vi "Host Image Acquisition Module.vi"(8 "error in":errorcluster, 11 "Operation":T3) -> (0 "error out":errorcluster, 1 "Image Acquired":bool, 2 "Acq In Progress":bool, 3 "Image":T2(plugin-control))   [LabVIEW 2013]
uses:
  Host Image Acquisition Module Enum.ctl
  Acquisition Settings Cluster.ctl
  <vilib>/vision/Image Controls.llb/IMAQ Image.ctl
  Common/CL Configuration.ctl
  Common/CL Signal Mapping.ctl
  Image Acquisition Settings FG Enum.ctl
  System Status/Status FG Enum.ctl
  Image Processing/Mask ROI FG Enum.ctl
  <vilib>/rvi/interface/common/niFpgaWaitOnOcc.vi
  <vilib>/FPGAPlugInAG/PCIe-1473R/niLvFpga_Reset_PCIe-1473R.vi
  <vilib>/Utility/error.llb/Error Cluster From Error Code.vi
  <vilib>/rvi/errors/niLvFpgaAdjustHostInterfaceError.vi
  <vilib>/FPGAPlugInAG/PCIe-1473R/niLvFpga_Run_PCIe-1473R.vi
  <vilib>/FPGAPlugInAG/PCIe-1473R/niLvFpga_Close_PCIe-1473R.vi
  <vilib>/rvi/interface/nirviMethod/nirviMethod.xnode
  FGs/FPGA_Reference.ctl
  8-Tap 8-bit Camera with DRAM Example/FPGA Bitfiles/8-Tap8-bitCamera_FPGATarget_8-Tap8-bit.lvbitx
  <vilib>/rvi/interface/nirviReadWriteControl/nirviReadWriteControl.xnode
  <vilib>/rvi/interface/nirviCloseFPGA/nirviCloseFPGA.xnode
  Common/Timing/Timing Lib.lvlib
  Globals/Average Sector Data.vi
  <vilib>/rvi/errors/niLvFpgaMergeErrorWithErrorCode.vi
  NiFpgaLv.dll
  <vilib>/FPGAPlugInAG/PCIe-1473R/niLvFpga_ReadFifo_PCIe-1473R.vi
  <vilib>/FPGAPlugInAG/PCIe-1473R/niLvFpga_ConfigureFifo_PCIe-1473R.vi
  <vilib>/FPGAPlugInAG/PCIe-1473R/niLvFpga_StartFifo_PCIe-1473R.vi
panel:
  out "Frames To Acquire":u32
  out "Image Height":u32
  out "Actual Depth":u32
  out "Target Sim TO":bool
  out "Cam Data Timeout":bool
  out "Sector FIFO Timeout":bool
  out "Host DMA Timeout":bool
  out "Number of Elements to Write Host DMA":u32
  out "Number of Elements to Read Cam Data":u32
  out "Image Data":u64[](array[numeric])
  out "Elements Remaining":u32
  out "Words per image":u32
  out "Num Frames read":u32
  out "DMA Words per Image":u32
  out "Acquire":bool
  in  "Acquisition Settings Cluster":T1={"Image Width"=1200, "Image Height"=788, "Frames To Acquire"=0, "Signal Mapping"=enum."Standard", "DMA Buffer Size\n(In Images)"=64} {"Image Height" max=65535; "Image Width" max=65535 step=40}
  out "Buffer Size":u32
  out "Acq'd Frame Width":u32=2040
  out "DMA Write Timeout":bool
  in  "Start Serial Server":bool
  out "Frames Acq'd":u32=1
  out "Acq'd Frame Height":u32=1088
  out "Initialized":bool
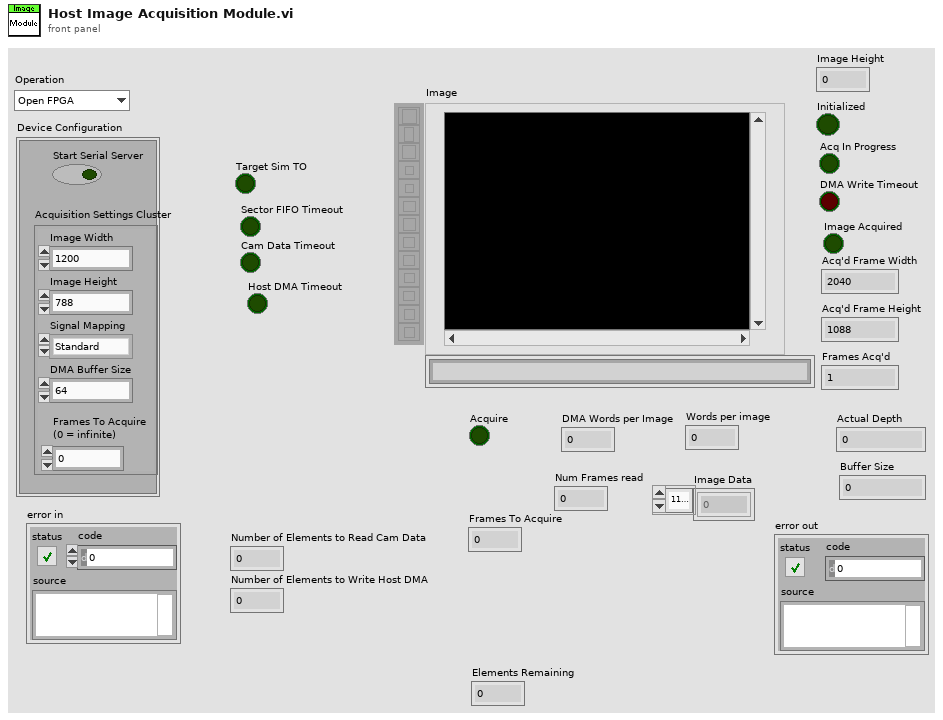
[diagram p1: front panel]
types:
  T1 = typedef "Acquisition Settings Cluster.ctl" = cluster{"Image Width":u32, "Image Height":u32, "Frames To Acquire":u32, "Signal Mapping":enum8{"Standard", "Basler 10-tap", "Vosskühler 10-tap"}, "DMA Buffer Size\n(In Images)":u32}
  T2 = typedef "IMAQ Image.ctl" = refnum<image>
  T3 = typedef "Host Image Acquisition Module Enum.ctl" = enum16{"Open FPGA", "Initialize DMA FIFO", "Load Sim Images", "Initialize Acquisition", "Update Sector Parameters", "Start Acquisition", "Aquire Image", "Read Averages", "Cancel Acquisition", "Close FPGA"}
  T4 = typedef "Image Acquisition Settings FG Enum.ctl" = enum16{"Read", "Write"}
  T5 = typedef "CL Signal Mapping.ctl" = enum8{"Standard", "Basler 10-tap", "Vosskühler 10-tap"}
  T6 = typedef "CL Configuration.ctl" = enum8{"Base", "Medium", "Full"}
  T7 = typedef "Status FG Enum.ctl" = enum16{"Reset", "Read", "Write"}
  T8 = typedef "Mask ROI FG Enum.ctl" = enum16{"Read", "Write"}
  T9 = enum16{"big-endian, network order", "native, host order", "little-endian"}
  T10 = typedef "FPGA_Reference.ctl" = refnum<k20>
  T11 = typedef "Image Type" = u32
  T12 = typedef "Mask ROI Cluster.ctl" = cluster{"left annulus":T13, "right annulus":T13, "Threshold Range":cluster{"Lower value":dbl, "Upper value":dbl}, "[Avg BG]":u8[], "Number of Sectors":u8, "Left ROI":T14, "Right ROI":T14, "Left Start Angle Duty Cycle":fxp<+,8,0>, "Left End Angle Duty Cycle":fxp<+,8,0>, "Right End Angle Duty Cycle":fxp<+,8,0>, "Right Start Angle Duty Cycle":fxp<+,8,0>, "[Sector ROIs]":T14[]}
  T13 = typedef "IMAQ Circle" = cluster{"Center X":i32, "Center Y":i32, "Inner Radius":i32, "Outer Radius":i32, "Start Angle":dbl, "End Angle":dbl}
  T14 = typedef "ROI Descriptor" = cluster{"Global Rectangle":i32[], "Contours":cluster{"ID":enum32{"External", "Internal"}, "Type":u32, "Coordinates":i32[]}[]}
  T15 = typedef "Sector Parameter Cluster.ctl" = cluster{"Start Angle":fxp<+/-,17,2>, "End Angle":fxp<+,17,3>, "Inner Radius":u16, "Outter Radius":u16, "Hinge X":u16, "Hinge Y":u16, "NumWingSectors":u8}
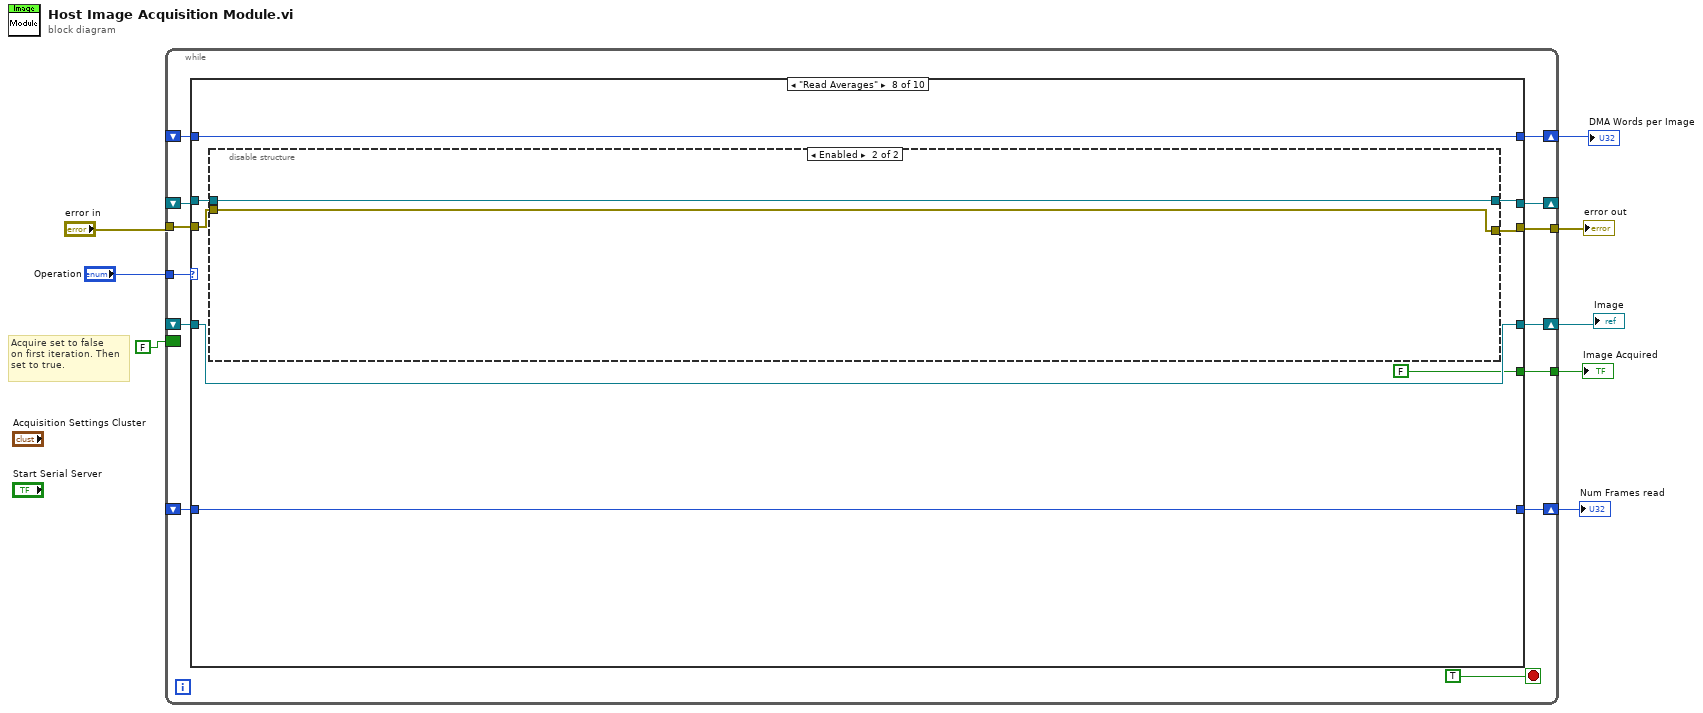
[diagram p0: block diagram]
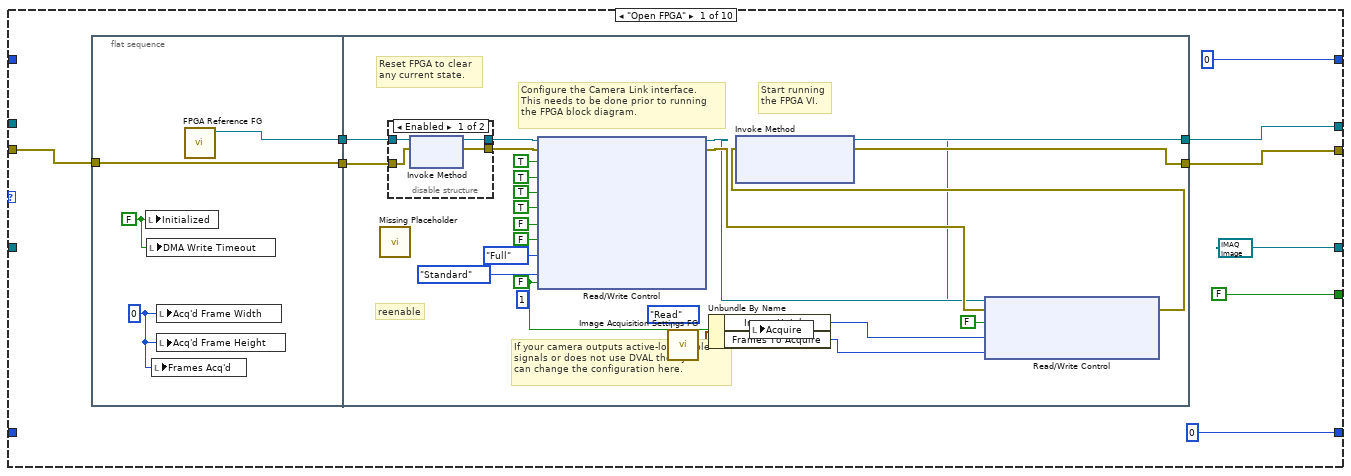
[diagram p2: hidden frame]
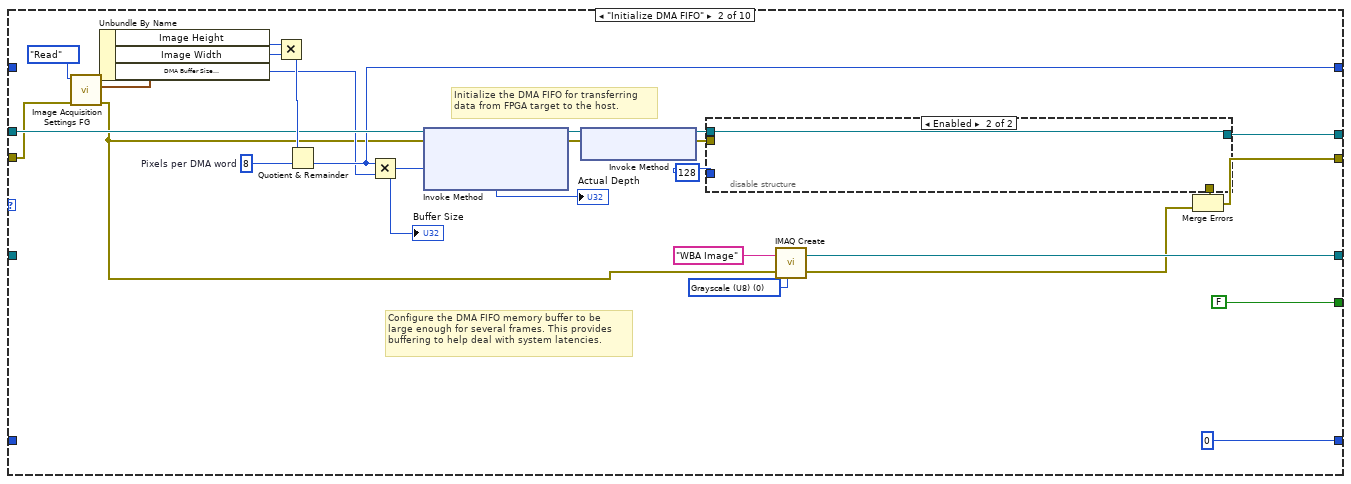
[diagram p4: hidden frame]
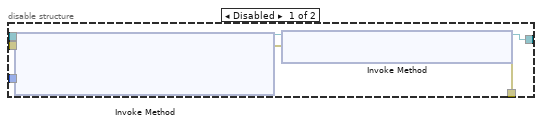
[diagram p5: hidden frame]
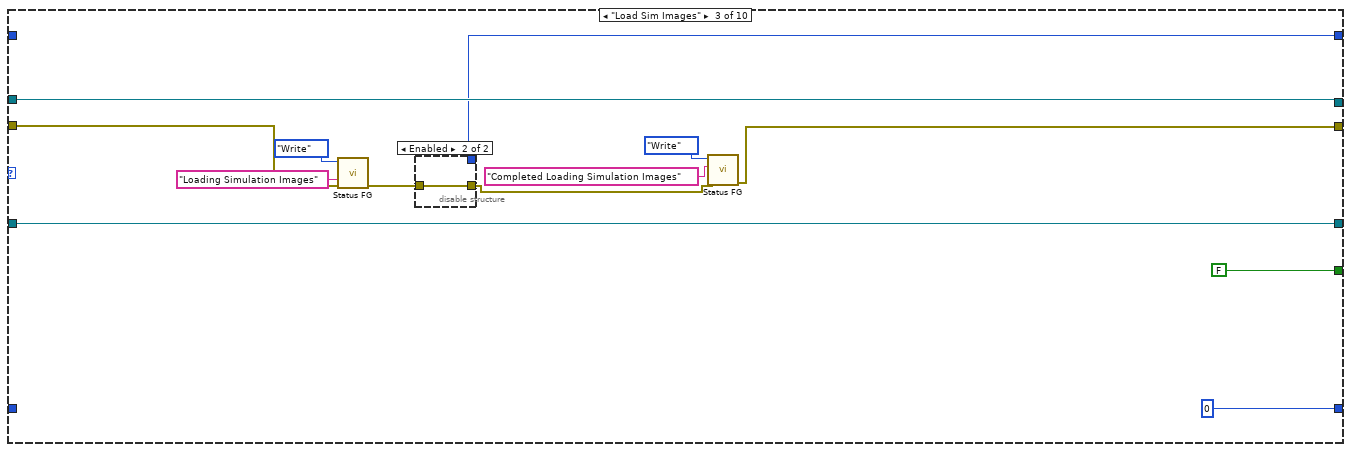
[diagram p6: hidden frame]
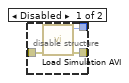
[diagram p7: hidden frame]
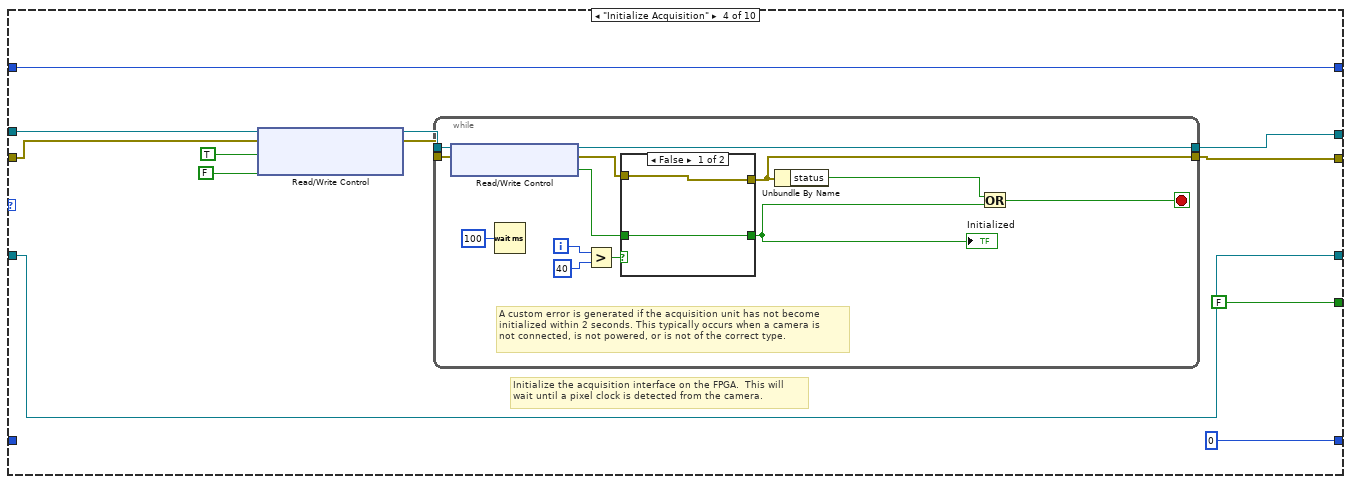
[diagram p8: hidden frame]
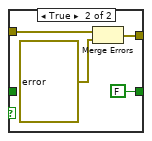
[diagram p9: hidden frame]
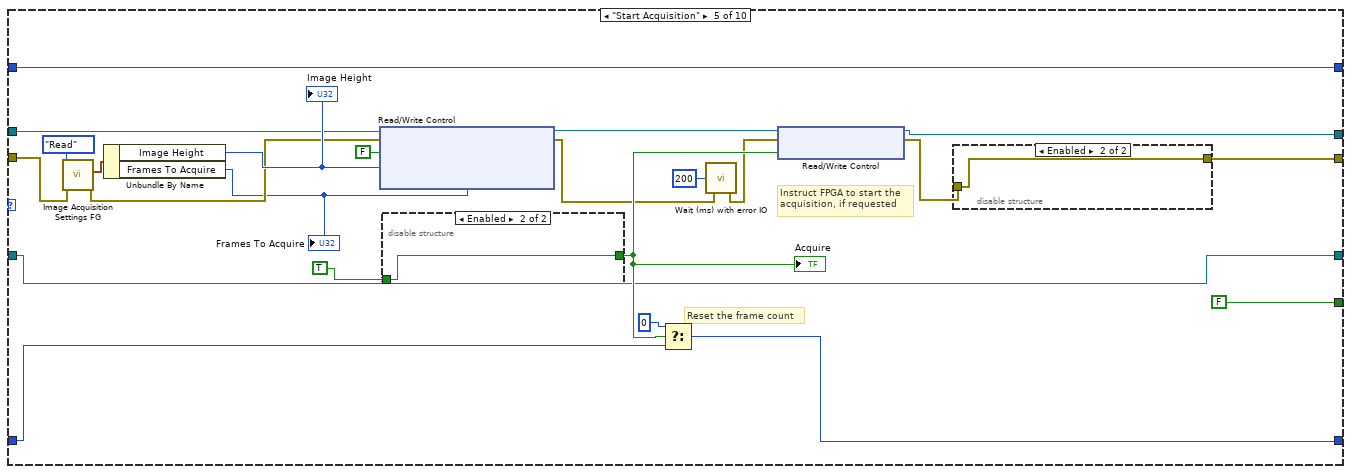
[diagram p10: hidden frame]
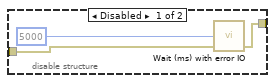
[diagram p11: hidden frame]
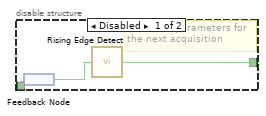
[diagram p12: hidden frame]
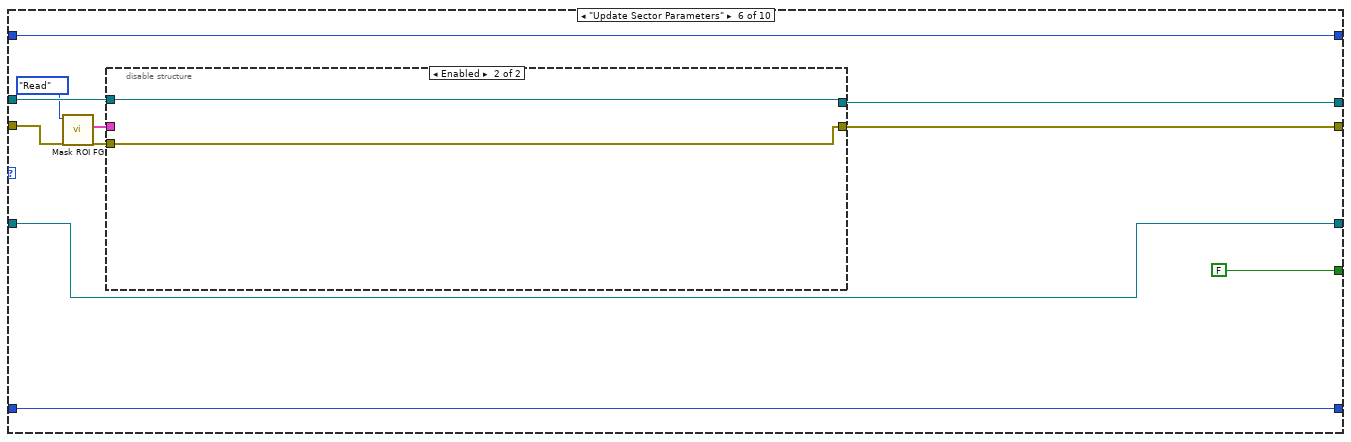
[diagram p13: hidden frame]
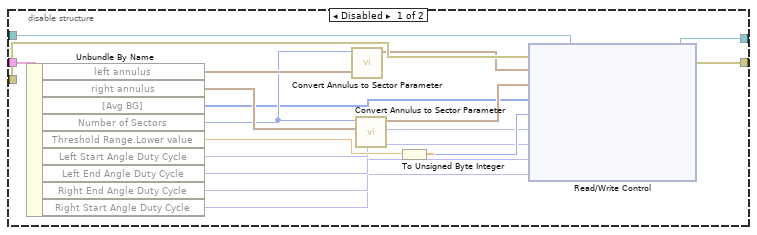
[diagram p14: hidden frame]
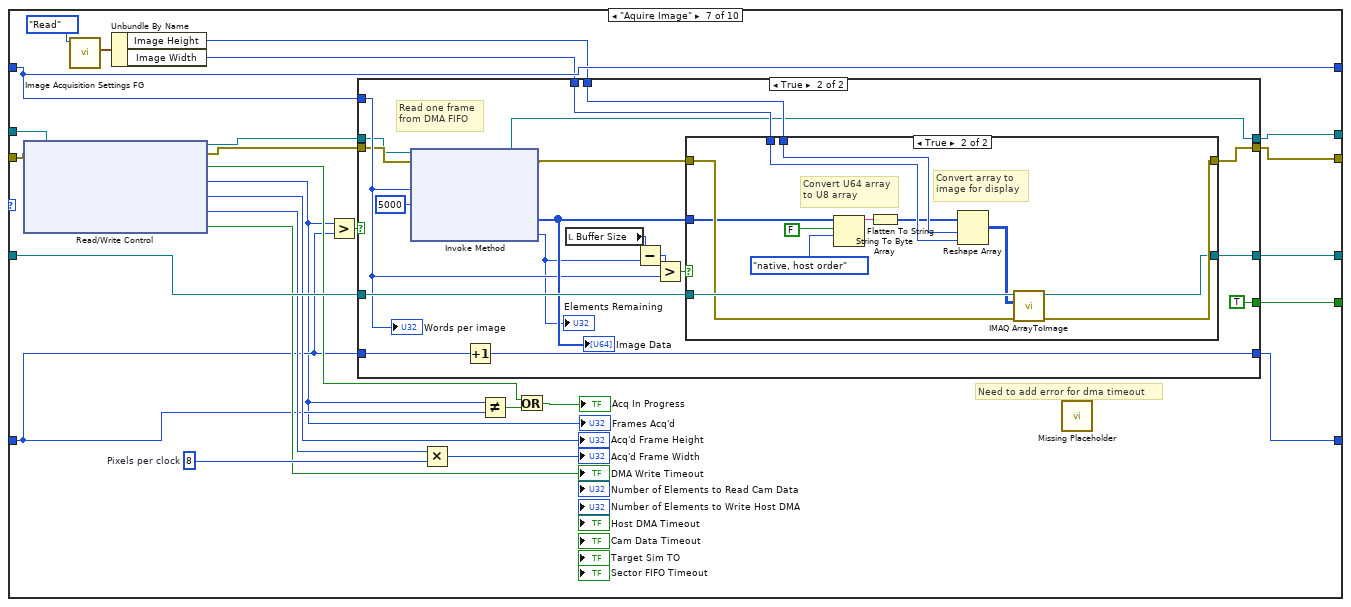
[diagram p15: hidden frame]
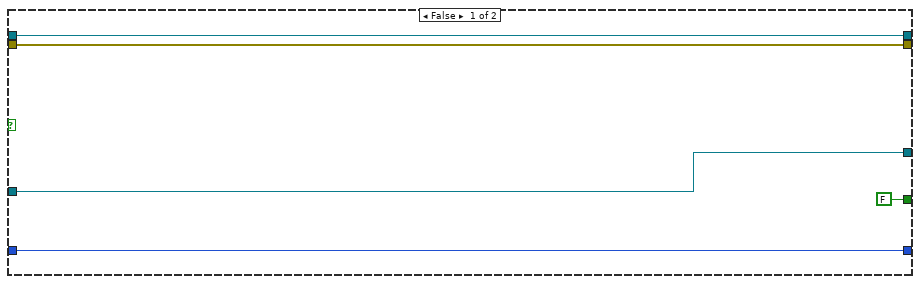
[diagram p16: hidden frame]
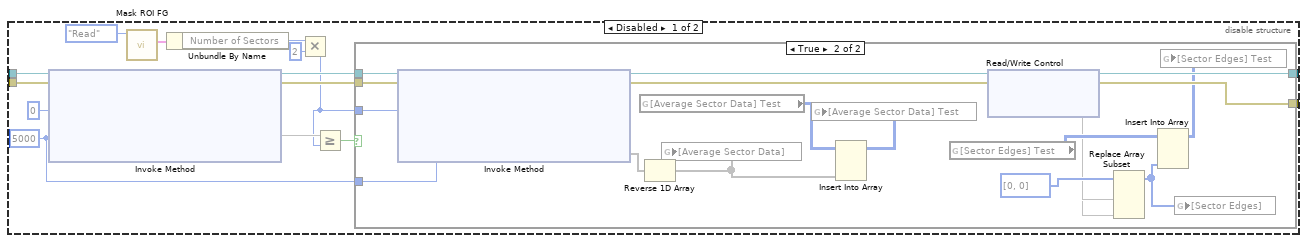
[diagram p18: hidden frame]
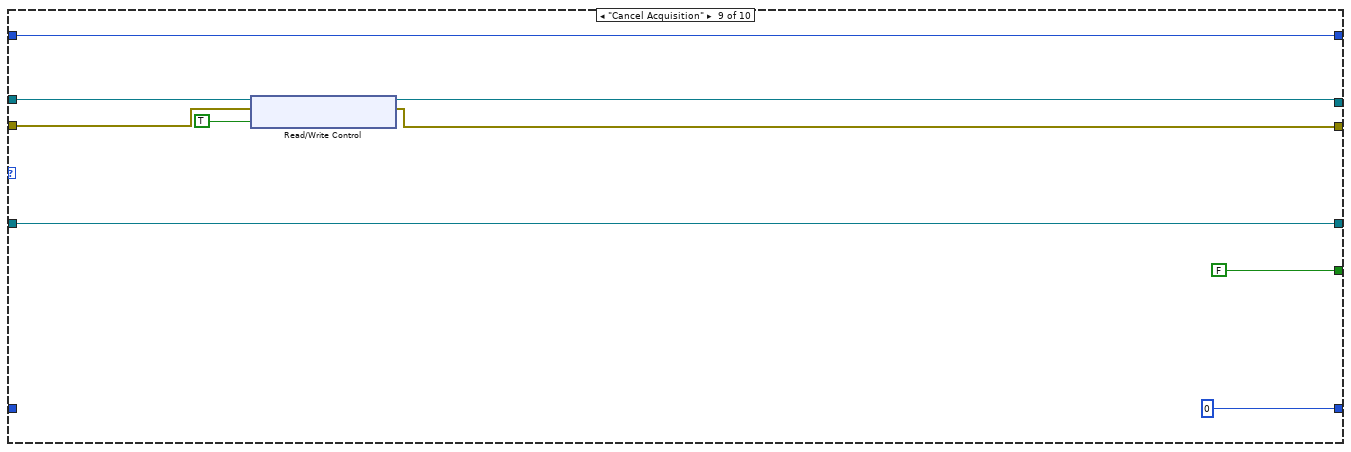
[diagram p20: hidden frame]
diagram:
  # "Acquire set to false\non first iteration. Then\nset to true."
  n1 = while {
    shift-right: [w20] -> _
    shift-left: _ -> [w16]
    tunnel: "error in" -> [w19]
    tunnel: "Operation" -> [w18]
    tunnel: [w17] -> w6
    shift-right: [w15] -> w3
    shift-left: _ -> [w14]
    shift-right: [w13] -> w4
    shift-left: _ -> [w10]
    shift-right: [w12] -> w2
    shift-left: _ -> [w11]
    border: FALSE ("Acquire") -> [_]
    tunnel: [w9] -> w1
    stop <- TRUE stop-if-true
    n2 = case shown="\"Read Averages\"" w18 {
      tunnel: w19 -> [w30 w78 w107 w118 w163 w187 w215 w273 w322 w328]
      tunnel: [w29 w70 w110 w124 w156 w183 w233 w279 w324 w329] -> w20
      tunnel: [w28 w71 w101 w120 w154 w184 w232 w274 w321 w335] -> w17
      tunnel: w16 -> [_ w86 w110 w125 w164 w189 w234 w280 w326 w331]
      tunnel: [u32 0 w85 w109 w123 w159 w188 w225 w278 w320 w332] -> w15
      tunnel: w14 -> [_ _ _ w123 w159 w188 w225 w278 w320 w332]
      tunnel: [T2 refnum ("New Image") w81 w111 w119 w158 w180 w227 w277 w323 w333] -> w13
      tunnel: [u32 0 u32 0 u32 0 u32 0 w160 w182 w231 w276 u32 0 w334] -> w12
      tunnel: w11 -> [_ _ _ _ w161 w182 w213 w276 _ w334]
      tunnel: w10 -> [_ _ w111 w119 w158 w180 w226 w277 w323 w333]
      tunnel: [FALSE ("Image Acquired") FALSE ("Image Acquired") FALSE ("Image Acquired") FALSE ("Image Acquired") FALSE ("Image Acquired") FALSE ("Image Acquired") w209 FALSE ("Image Acquired") FALSE ("Image Acquired") FALSE ("Image Acquired")] -> w9
      frame "Open FPGA" {
        n3 = flat-sequence {
          tunnel: w30 -> [w31]
          tunnel: [w32] -> w27
          tunnel: [w31] -> w26
          tunnel: [w47] -> w28
          tunnel: [w48] -> w29
          tunnel: w27 -> [w51]
          tunnel: w26 -> [w49]
          frame #0 {
            w33 = u32 0 ("Acq'd Frame Width")
            w34 = FALSE ("Initialized")
            n4 = local write "Initialized"(w34) -> ()
            n5 = local write "DMA Write Timeout"(w34) -> ()
            n6 = local write "Frames Acq'd"(w33) -> ()
            n7 = local write "Acq'd Frame Width"(w33) -> ()
            n8 = local write "Acq'd Frame Height"(w33) -> ()
            n9 = call "FPGA Reference FG.vi"() -> ("FPGA VI Reference Out"=w32:T10)  [unwired: 11 in]
          }
          frame #1 {
            (unwired) u8 1 ("# of Frames to Average")
            w46 = FALSE ("Acq Control.Acquire")
            # "reenable"
            # "If your camera outputs active-low enable\nsignals or does not use DVAL then you \ncan change the configuration here."
            # "Start running\nthe FPGA VI."
            # "Reset FPGA to clear\nany current state."
            # "Configure the Camera Link interface.\nThis needs to be done prior to running\nthe FPGA block diagram."
            n10 = call "Missing Placeholder.vi"() -> ()  [unwired: 12 in]
            n11 = disable-structure shown="Enabled" {
              disable-tunnel: [w62 w64] -> w53
              disable-tunnel: [w61 w63] -> w52
              disable-tunnel: w51 -> [w60 w64]
              disable-tunnel: w49 -> [w59 w63]
              frame Enabled {
                n12 = xnode "Invoke Method"("FPGA VI Reference In"=w60, "error in"=w59) -> ("FPGA VI Reference Out"=w62:T10, "error out"=w61:errorcluster)
              }
              frame Disabled {
              }
            }
            n13 = xnode "Read/Write Control"("FPGA VI Reference In"=w53, "error in"=w52, "CL Config.FVAL Active High"=TRUE ("IO Module Config.CL FVAL Active High"), "CL Config.LVAL Active High"=TRUE ("IO Module Config.CL LVAL Active High"), "CL Config.DVAL Active High"=TRUE ("IO Module Config.CL DVAL Active High"), "CL Config.Spare Active High"=TRUE ("IO Module Config.CL Spare Active High"), "CL Config.Line Scan"=FALSE, "Acq Control.Ignore DVAL"=FALSE ("CL Config.Line Scan"), "CL Config.Configuration"=CL_Configuration."Full", "CL Config.Signal Mapping"=CL_Signal_Mapping."Standard", "Acq Control.Acquire"=w46) -> ("FPGA VI Reference Out"=w36:T10, "error out"=w38:errorcluster)
            n14 = call "Image Acquisition Settings FG.vi"("Operation"=Image_Acquisition_Settings_FG_Enum."Read") -> ("Acquisition Settings Out"=w43:T1)  [unwired: 9 in, 1 out]
            n15 = Unbundle By Name(w43) -> ("Image Height"=w41:u32, "Frames To Acquire"=w39:u32)
            n16 = local write "Acquire"(w46) -> ()
            n17 = xnode "Read/Write Control"("FPGA VI Reference In"=w36, "error in"=w38, "Acq Control.Cancel Acq"=FALSE, "Acq Control.Line Scan Height"=w41, "Acq Control.Frames To Acq"=w39) -> ("FPGA VI Reference Out"=w35:T10, "error out"=w37:errorcluster)
            n18 = xnode "Invoke Method"("FPGA VI Reference In"=w35, "error in"=w37) -> ("FPGA VI Reference Out"=w48:T10, "error out"=w47:errorcluster)  [unwired: 1 in]
          }
        }
      }
      frame "Initialize DMA FIFO" {
        w82 = T11 0 items=["Grayscale (U8)", "Grayscale (I16)", "Grayscale (SGL)", "Complex (CSG)", "RGB (U32)", "HSL (U32)", "RGB (U64)", "Grayscale (U16)"] ("Image Type")
        w88 = u32 8  # Pixels per DMA word
        # "Configure the DMA FIFO memory buffer to be\nlarge enough for several frames. This provides\nbuffering to help deal with system latencies."
        # "Initialize the DMA FIFO for transferring\ndata from FPGA target to the host."
        n19 = call "Image Acquisition Settings FG.vi"("error in (no error)"=w78, "Operation"=Image_Acquisition_Settings_FG_Enum."Read") -> ("error out"=w73:errorcluster, "Acquisition Settings Out"=w79:T1)  [unwired: 8 in]
        n20 = Unbundle By Name(w79) -> ("Image Height"=w77:u32, "Image Width"=w76:u32, "DMA Buffer Size\n(In Images)"=w75:u32)
        n21 = Multiply(x=w77, y=w76) -> (x*y=w87:u32)
        n22 = Quotient & Remainder(x=w87, y=w88) -> (floor(x/y)=w85:u32)  [unwired: 1 out]
        n23 = Multiply(x=w85, y=w75) -> (x*y=w89:u32)
        "Buffer Size" <- w89
        n24 = xnode "Invoke Method"("FPGA VI Reference In"=w86, "error in"=w73, "Requested Depth"=w89) -> ("FPGA VI Reference Out"=w91:T10, "error out"=w90:errorcluster, "Actual Depth"=→"Actual Depth":u32)
        n25 = xnode "Invoke Method"("FPGA VI Reference In"=w91, "error in"=w90) -> ("FPGA VI Reference Out"=w68:T10, "error out"=w66:errorcluster)
        n26 = disable-structure shown="Enabled" {
          disable-tunnel: u32 128 ("Requested Depth") -> [w98 _]
          disable-tunnel: [w97 w99] -> w70
          disable-tunnel: w68 -> [w96 w99]
          disable-tunnel: w66 -> [w95 _]
          disable-tunnel: [w92 _] -> w65
          frame Disabled {
            n27 = xnode "Invoke Method"("FPGA VI Reference In"=w96, "error in"=w95, "Requested Depth"=w98) -> ("FPGA VI Reference Out"=w94:T10, "error out"=w93:errorcluster)  [unwired: 1 out]
            n28 = xnode "Invoke Method"("FPGA VI Reference In"=w94, "error in"=w93) -> ("FPGA VI Reference Out"=w97:T10, "error out"=w92:errorcluster)
          }
          frame Enabled {
          }
        }
        n29 = call "IMAQ Create"("Image Name"="WBA Image", "Image Type"=w82, "error in (no error)"=w73) -> ("New Image"=w81:T2, "error out"=w72:errorcluster)  [unwired: 2 in]
        n30 = Merge Errors(w65, w72) -> (w71:errorcluster)
      }
      frame "Load Sim Images" {
        n31 = call "Status FG.vi"("error in (no error)"=w107, "Status In"="Loading Simulation Images", "Operation"=Status_FG_Enum."Write") -> ("error out"=w106:errorcluster)  [unwired: 7 in, 1 out]
        n32 = disable-structure shown="Enabled" {
          disable-tunnel: [w115 _] -> w109
          disable-tunnel: w106 -> [w114 w116]
          disable-tunnel: [w113 w116] -> w102
          frame Disabled {
            n33 = call "Load Simulation AVI.vi"("error in (no error)"=w114) -> ("error out"=w113:errorcluster, "Words per image"=w115:u32)  [unwired: 9 in]
          }
          frame Enabled {
          }
        }
        n34 = call "Status FG.vi"("error in (no error)"=w102, "Status In"="Completed Loading Simulation Images", "Operation"=Status_FG_Enum."Write") -> ("error out"=w101:errorcluster)  [unwired: 7 in, 1 out]
      }
      frame "Initialize Acquisition" {
        # "Initialize the acquisition interface on the FPGA.  This will\nwait until a pixel clock is detected from the camera."
        n35 = xnode "Read/Write Control"("FPGA VI Reference In"=w125, "error in"=w118, "Acq Control.Initialize"=TRUE ("Arm Acquisition"), "Acq Control.Cancel Acq"=FALSE) -> ("FPGA VI Reference Out"=w128:T10, "error out"=w127:errorcluster)
        n36 = while {
          tunnel: w128 -> [w137]
          tunnel: w127 -> [w136]
          tunnel: [w135] -> w124
          tunnel: [w138] -> w120
          i -> [w131]
          stop <- w141 stop-if-true
          # "A custom error is generated if the acquisition unit has not become\ninitialized within 2 seconds. This typically occurs when a camera is\nnot connected, is not powered, or is not of the correct type."
          n37 = xnode "Read/Write Control"("FPGA VI Reference In"=w137, "error in"=w136) -> ("FPGA VI Reference Out"=w135:T10, "error out"=w134:errorcluster, "Acq Status.Initialized"=w133:bool)
          n38 = Wait (ms)(milliseconds to wait=u32 100) -> ()  [unwired: 1 out]
          n39 = Greater?(x=w131, y=40) -> (0:w132:bool)
          n40 = case shown="False" w132 {
            tunnel: [w143 FALSE] -> w129
            tunnel: w133 -> [w143 _]
            tunnel: w134 -> [w142 w145]
            tunnel: [w142 w147] -> w138
            frame False {
            }
            frame True {
              n41 = Merge Errors(w145, errorcluster {"status"=TRUE, "code"=-8999, "source"="Acquisition Initialization: This error typically occurs when a camera is not properly connected, is not powered, or is not of the correct type."} ("error in")) -> (w147:errorcluster)
            }
          }
          "Initialized" <- w129
          n42 = Unbundle By Name(w138) -> ("status"=w140:bool)
          n43 = Or(x=w140, y=w129) -> (x .or. y?=w141:bool)
        }
      }
      frame "Start Acquisition" {
        # "Reset the frame count"
        # "Instruct FPGA to start the\nacquisition, if requested"
        n44 = call "Image Acquisition Settings FG.vi"("error in (no error)"=w163, "Operation"=Image_Acquisition_Settings_FG_Enum."Read") -> ("error out"=w162:errorcluster, "Acquisition Settings Out"=w170:T1)  [unwired: 8 in]
        n45 = Unbundle By Name(w170) -> ("Image Height"=w165:u32, "Frames To Acquire"=w152:u32)
        "Image Height" <- w165
        "Frames To Acquire" <- w152
        n46 = xnode "Read/Write Control"("FPGA VI Reference In"=w164, "error in"=w162, "Acq Control.Cancel Acq"=FALSE, "Acq Control.Line Scan Height"=w165, "Acq Control.Frames To Acq"=w152) -> ("FPGA VI Reference Out"=w151:T10, "error out"=w150:errorcluster)
        n47 = disable-structure shown="Enabled" {
          disable-tunnel: [w177 w178] -> w167
          disable-tunnel: TRUE ("Acquire") -> [w175 w178]
          frame Disabled {
            # "Write the parameters for\nthe next acquisition"
            n48 = feedback #1() -> (w176:bool)
            n49 = feedback-in #1(w175) -> ()
            n50 = call "Rising Edge Detect.vi"("Input"=w176) -> ("Pulse"=w177:bool)  [unwired: 4 in]
          }
          frame Enabled {
          }
        }
        "Acquire" <- w167
        n51 = Select(t=u32 0, s=w167, f=w161) -> (s? t:f=w160:u32)
        n52 = call "Wait (ms) with error IO.vi"("error in (no error)"=w150, "milliseconds to wait"=u32 200) -> ("error out"=w149:errorcluster)  [unwired: 3 in]
        n53 = xnode "Read/Write Control"("FPGA VI Reference In"=w151, "error in"=w149, "Acq Control.Acquire"=w167) -> ("FPGA VI Reference Out"=w156:T10, "error out"=w155:errorcluster)
        n54 = disable-structure shown="Enabled" {
          disable-tunnel: w155 -> [w172 w174]
          disable-tunnel: [w171 w174] -> w154
          frame Disabled {
            n55 = call "Wait (ms) with error IO.vi"("error in (no error)"=w172, "milliseconds to wait"=u32 5000) -> ("error out"=w171:errorcluster)  [unwired: 3 in]
          }
          frame Enabled {
          }
        }
      }
      frame "Update Sector Parameters" {
        n56 = call "Mask ROI FG.vi"("error in (no error)"=w187, "Operation"=Mask_ROI_FG_Enum."Read") -> ("error out"=w186:errorcluster, "Mask ROI Out"=w181:T12)  [unwired: 8 in]
        n57 = disable-structure shown="Enabled" {
          disable-tunnel: w189 -> [w206 w208]
          disable-tunnel: w186 -> [w205 w207]
          disable-tunnel: [w204 w207] -> w184
          disable-tunnel: [w203 w208] -> w183
          disable-tunnel: w181 -> [w202 _]
          frame Disabled {
            n58 = Unbundle By Name(w202) -> ("left annulus"=w201:T13, "right annulus"=w199:T13, "[Avg BG]"=w196:u8[], "Number of Sectors"=w198:u8, "Threshold Range.Lower value"=w195:dbl, "Left Start Angle Duty Cycle"=w193:fxp<+,8,0>, "Left End Angle Duty Cycle"=w192:fxp<+,8,0>, "Right End Angle Duty Cycle"=w191:fxp<+,8,0>, "Right Start Angle Duty Cycle"=w190:fxp<+,8,0>)
            n59 = call "Convert Annulus to Sector Parameter.vi"("Annulus"=w201, "NumWingSectors"=w198) -> ("Sector Parameter"=w200:T15)  [unwired: 9 in]
            n60 = call "Convert Annulus to Sector Parameter.vi"("Annulus"=w199, "NumWingSectors"=w198) -> ("Sector Parameter"=w197:T15)  [unwired: 9 in]
            n61 = To Unsigned Byte Integer(number=w195) -> (unsigned 8bit integer=w194:u8)
            n62 = xnode "Read/Write Control"("FPGA VI Reference In"=w206, "error in"=w205, "Sector Parameters Left"=w200, "Sector Parameters Right"=w197, "[Average BG Intensity]"=w196, "Sector Threshold"=w194, "Left Start Angle Duty Cycle"=w193, "Left End Angle Duty Cycle"=w192, "Right End Angle Duty Cycle"=w191, "Right Start Angle Duty Cycle"=w190) -> ("FPGA VI Reference Out"=w203:T10, "error out"=w204:errorcluster)
          }
          frame Enabled {
          }
        }
      }
      frame "Aquire Image" {
        w223 = u32 8  # Pixels per clock
        # "Need to add error for dma timeout"
        n63 = xnode "Read/Write Control"("FPGA VI Reference In"=w234, "error in"=w215) -> ("FPGA VI Reference Out"=w230:T10, "error out"=w229:errorcluster, "Acq Status.Acq In Progress"=w214:bool, "Acq Status.Frames Acq'd"=w212:u32, "Acq Status.Lines Per Frame"=→"Acq'd Frame Height":u32, "Acq Status.Clocks Per Line"=w222:u32, "Acq Status.DMA Write Timeout"=→"DMA Write Timeout":bool)
        "Frames Acq'd" <- w212
        n64 = call "Image Acquisition Settings FG.vi"("Operation"=Image_Acquisition_Settings_FG_Enum."Read") -> ("Acquisition Settings Out"=w218:T1)  [unwired: 9 in, 1 out]
        n65 = Unbundle By Name(w218) -> ("Image Height"=w217:u32, "Image Width"=w216:u32)
        n66 = Greater?(x=w212, y=w213) -> (0:w228:bool)
        n67 = case shown="True" w228 {
          tunnel: w230 -> [w238 w241]
          tunnel: w229 -> [w237 w242]
          tunnel: w217 -> [_ w258]
          tunnel: w216 -> [_ w257]
          tunnel: w226 -> [w239 w256]
          tunnel: [w237 w254] -> w232
          tunnel: [w238 w253] -> w233
          tunnel: w213 -> [w236 w252]
          tunnel: [w236 w251] -> w231
          tunnel: w225 -> [_ w248]
          tunnel: [w239 w247] -> w227
          tunnel: [FALSE ("Image Acquired") TRUE ("Image Acquired")] -> w209
          frame False {
          }
          frame True {
            # "Read one frame\nfrom DMA FIFO"
            n68 = xnode "Invoke Method"("FPGA VI Reference In"=w241, "error in"=w242, "Number of Elements"=w248, "Timeout (ms)"=5000) -> ("FPGA VI Reference Out"=w253:T10, "error out"=w255:errorcluster, "Data"=w250:u64[], "Elements Remaining"=w245:u32)
            "Elements Remaining" <- w245
            "Image Data" <- w250
            n69 = Increment(x=w252) -> (x+1=w251:u32)
            n70 = local read "Buffer Size"() -> (w246:u32)
            n71 = Subtract(x=w246, y=w245) -> (x-y=w244:u32)
            n72 = Greater?(x=w244, y=w248) -> (0:w249:bool)
            n73 = case shown="True" w249 {
              tunnel: w258 -> [_ w272]
              tunnel: w257 -> [_ w271]
              tunnel: w256 -> [w259 w270]
              tunnel: w255 -> [w260 w269]
              tunnel: [w260 w268] -> w254
              tunnel: w250 -> [_ w265]
              tunnel: [w259 w261] -> w247
              frame False {
                # "Do not display the image if we're\nfalling behind in the acquisition."
              }
              frame True {
                # "Convert U64 array\nto U8 array"
                # "Convert array to\nimage for display"
                n74 = Flatten To String(anything=w265, prepend array or string size? (T)=FALSE, byte order (0:big-endian, network order)=T9."native, host order") -> (data string=w263:string)  [unwired: 1 in, 2 out]
                n75 = String To Byte Array(string=w263) -> (unsigned byte array=w262:u8[])
                n76 = Reshape Array(w262, w272, w271) -> (w267:u8[][])
                n77 = call "IMAQ ArrayToImage"("error in (no error)"=w269, "Image Pixels (U8)"=w267, "Image"=w270) -> ("error out"=w268:errorcluster, "Image Out"=w261:T2)  [unwired: 7 in]
              }
            }
            "Words per image" <- w248
          }
        }
        n78 = Multiply(x=w222, y=w223) -> (x*y=→"Acq'd Frame Width":u32)
        n79 = Not Equal?(x=w212, y=w213) -> (x != y?=w211:bool)
        n80 = Or(x=w214, y=w211) -> (x .or. y?=→"Acq In Progress":bool)
        n81 = call "Missing Placeholder.vi"() -> ()  [unwired: 12 in]
      }
      frame "Read Averages" {
        n82 = disable-structure shown="Enabled" {
          disable-tunnel: w280 -> [w295 w317]
          disable-tunnel: [w294 w317] -> w279
          disable-tunnel: [w293 w316] -> w274
          disable-tunnel: w273 -> [w292 w316]
          frame Disabled {
            w288 = 5000 ("Timeout (ms)")
            n83 = xnode "Invoke Method"("FPGA VI Reference In"=w295, "error in"=w292, "Number of Elements"=u32 0, "Timeout (ms)"=w288) -> ("FPGA VI Reference Out"=w290:T10, "error out"=w289:errorcluster, "Elements Remaining"=w283)  [unwired: 1 out]
            n84 = call "Mask ROI FG.vi"("Operation"=Mask_ROI_FG_Enum."Read") -> ("Mask ROI Out"=w286:T12)  [unwired: 9 in, 1 out]
            n85 = Unbundle By Name(w286) -> ("Number of Sectors"=w284:u8)
            n86 = Multiply(x=w284, y=u8 2) -> (x*y=w282:u8)
            n87 = Greater Or Equal?(x=w283, y=w282) -> (x >= y?=w285:bool)
            n88 = case shown="True" w285 {
              tunnel: w290 -> [w297 w315]
              tunnel: w289 -> [w296 w314]
              tunnel: w288 -> [_ w313]
              tunnel: [w297 w306] -> w294
              tunnel: [w296 w307] -> w293
              tunnel: w282 -> [_ w312]
              frame False {
              }
              frame True {
                n89 = xnode "Invoke Method"("FPGA VI Reference In"=w315, "error in"=w314, "Number of Elements"=w312, "Timeout (ms)"=w313) -> ("FPGA VI Reference Out"=w309:T10, "error out"=w308:errorcluster, "Data"=w303:void[])  [unwired: 1 out]
                n90 = global read "Average Sector Data.vi" "[Average Sector Data] Test"() -> (w311:u8[][])
                n91 = Reverse 1D Array(array=w303) -> (reversed array=w302:void[])
                n92 = global write "Average Sector Data.vi" "[Average Sector Data]"(w302) -> ()
                n93 = Insert Into Array(array=w311, new element=w302) -> (w310:u8[][])  [unwired: 2 in]
                n94 = global write "Average Sector Data.vi" "[Average Sector Data] Test"(w310) -> ()
                n95 = global read "Average Sector Data.vi" "[Sector Edges] Test"() -> (w305:u8[][])
                n96 = xnode "Read/Write Control"("FPGA VI Reference In"=w309, "error in"=w308) -> ("FPGA VI Reference Out"=w306:T10, "error out"=w307:errorcluster, "Right Sector Edge"=w300, "Left Sector Edge"=w299)
                n97 = Replace Array Subset(array=u8[] [0, 0] ("[Sector Edges]"), new element #1=w300, new element #2=w299) -> (w298:u8[])  [unwired: 2 in]
                n98 = Insert Into Array(array=w305, new element=w298) -> (w304:u8[][])  [unwired: 2 in]
                n99 = global write "Average Sector Data.vi" "[Sector Edges] Test"(w304) -> ()
                n100 = global write "Average Sector Data.vi" "[Sector Edges]"(w298) -> ()
              }
            }
          }
          frame Enabled {
          }
        }
      }
      frame "Cancel Acquisition" {
        n101 = xnode "Read/Write Control"("FPGA VI Reference In"=w326, "error in"=w322, "Acq Control.Cancel Acq"=TRUE) -> ("FPGA VI Reference Out"=w324:T10, "error out"=w321:errorcluster)
      }
      frame "Close FPGA" {
        n102 = xnode "Read/Write Control"("FPGA VI Reference In"=w331, "Acq Control.Cancel Acq"=TRUE) -> ("FPGA VI Reference Out"=w329:T10)  [unwired: 1 in, 1 out]
        n103 = xnode "Close FPGA VI Reference"("FPGA VI Reference In"=w329, "error in"=w328) -> ("error out"=w338:errorcluster)
        n104 = call <vilib>:"Simple Error Handler.vi"("error in (no error)"=w338) -> ("error out"=w336:errorcluster)  [unwired: 4 in, 4 out]
        n105 = call "IMAQ Dispose"("Image"=w333, "error in (no error)"=w336) -> ("error out"=w335:errorcluster)  [unwired: 4 in]
        n106 = local write "Initialized"(FALSE ("Initialized")) -> ()
      }
    }
  }
  "error out" <- w6
  "Image" <- w4
  "DMA Words per Image" <- w3
  "Num Frames read" <- w2
  "Image Acquired" <- w1
